vi "Func-yyllEnqueue.vi"(4 "Enable?(T)":bool=TRUE, 6 "data":variant, 7 "队列为空才入队（F）":bool, 8 "error in (no error)":errorcluster, 9 "timeout in ms (-1)":i32=-1, 10 "cmd":string, 11 "queue in":refnum<queue>) -> (0 "error out":errorcluster, 1 "timed out?":bool, 3 "queue out":refnum<queue>)   [LabVIEW 2017]
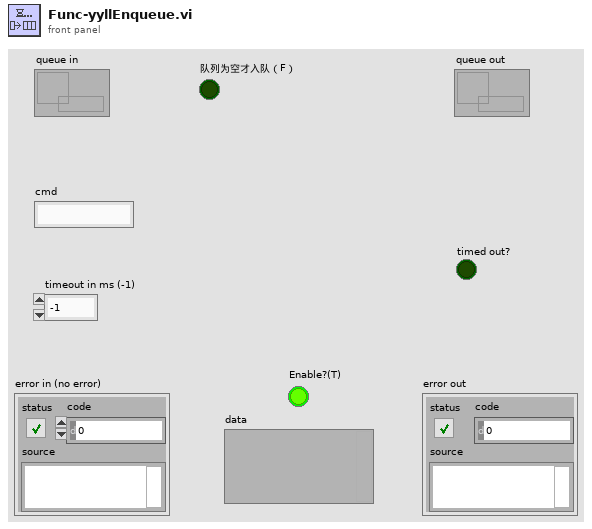
[diagram p1: front panel]
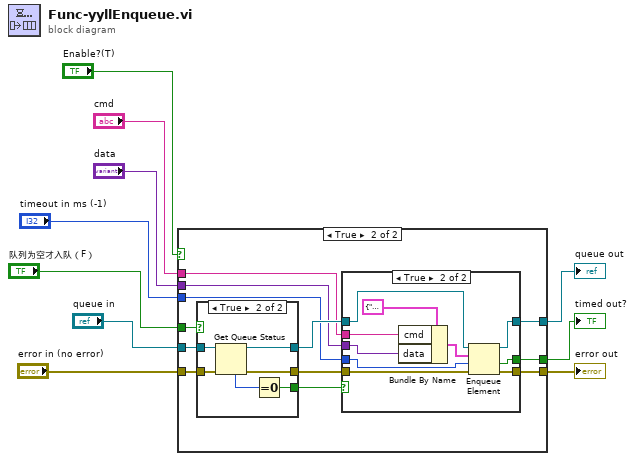
[diagram p0: block diagram]
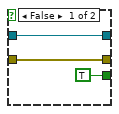
[diagram p4: hidden frame]
diagram:
  n1 = case shown="True" "Enable?(T)" {
    tunnel: "error in (no error)" -> [w12 w14]
    tunnel: [w12 w24] -> w9
    tunnel: "queue in" -> [w11 w22]
    tunnel: "队列为空才入队（F）" -> [_ w21]
    tunnel: "cmd" -> [_ w20]
    tunnel: "data" -> [_ w19]
    tunnel: "timeout in ms (-1)" -> [_ w18]
    tunnel: [w11 w16] -> w2
    tunnel: [_ w15] -> w1
    frame False {
    }
    frame True {
      n2 = case shown="True" w21 {
        tunnel: w22 -> [w38 w45]
        tunnel: [TRUE w43] -> w17
        tunnel: [w38 w42] -> w23
        tunnel: w14 -> [w37 w41]
        tunnel: [w37 w40] -> w13
        frame False {
        }
        frame True {
          n3 = Get Queue Status(queue=w45, error in (no error)=w41) -> (queue out=w42:refnum<queue>, error out=w40:errorcluster, # elements in queue=w44:i32)  [unwired: 1 in, 5 out]
          n4 = Equal To 0?(x=w44) -> (x = 0?=w43:bool)
        }
      }
      n5 = case shown="True" w17 {
        tunnel: [w26 w35] -> w16
        tunnel: w13 -> [w25 w33]
        tunnel: [_ w32] -> w15
        tunnel: [w25 w31] -> w24
        tunnel: w23 -> [w26 w30]
        tunnel: w20 -> [_ w29]
        tunnel: w19 -> [_ w28]
        tunnel: w18 -> [_ w27]
        frame False {
        }
        frame True {
          n6 = Bundle By Name(cluster=cluster{"cmd":string, "data":variant} {"cmd"="", "data"=variant} ("element"), "cmd"=w29, "data"=w28) -> (w34:cluster{"cmd":string, "data":variant})
          n7 = Enqueue Element(queue=w30, element=w34, timeout in ms (-1)=w27, error in (no error)=w33) -> (queue out=w35:refnum<queue>, timed out?=w32:bool, error out=w31:errorcluster)
        }
      }
    }
  }
  "error out" <- w9
  "queue out" <- w2
  "timed out?" <- w1
